vi "Set_Get_FVG.vi"(8 "error out":errorcluster, 9 "Tab Control":enum32{" START ", " HOME ", " TEST "}(ring), 10 "Message":T1=enum."Update Display", 11 "Enum":T2) -> (0 "error out 2":errorcluster, 2 "Tab Control 2":enum32{" START ", " HOME ", " TEST "}(ring), 3 "Message 2":T1)   [LabVIEW 2021]
uses:
  Control/Set_Get.ctl
  controls/test_sequence .ctl
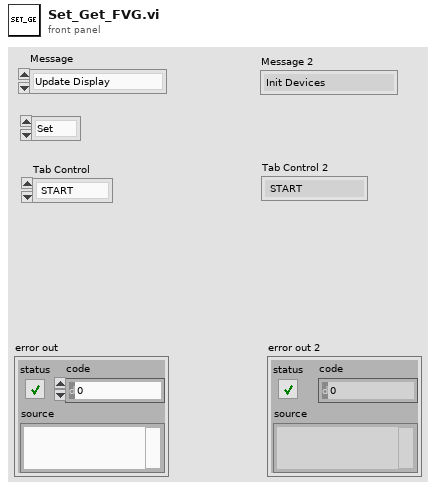
[diagram p1: front panel]
types:
  T1 = typedef "test_sequence .ctl" = enum16{"Init Devices", "Login", "Option Window", "Idle state", "Check", "Uncheck", "Scan Barcode", "Clear the test Containers", "Init-Pre Test", "Test ", "Result", "Report", "Database", "Update Display", "Confirm Quit", "Error", "Exit"}
  T2 = typedef "Set_Get.ctl" = enum16{"Set", "Get"}
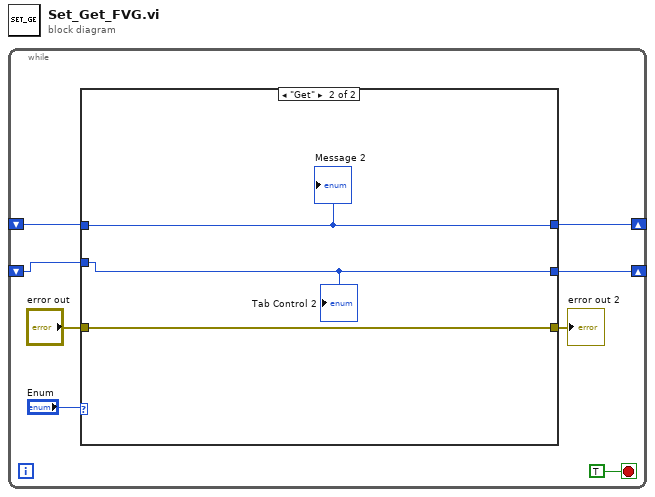
[diagram p0: block diagram]
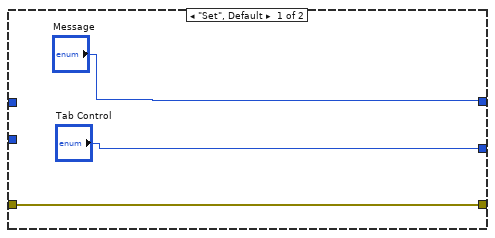
[diagram p2: hidden frame]
diagram:
  n1 = while {
    shift-right: [w7] -> _
    shift-left: _ -> [w6]
    shift-right: [w2] -> _
    shift-left: _ -> [w1]
    stop <- TRUE stop-if-true
    n2 = case shown="\"Get\"" "Enum" {
      tunnel: ["Message" w14] -> w7
      tunnel: w6 -> [_ w14]
      tunnel: [w10 w13] -> w3
      tunnel: "error out" -> [w10 w13]
      tunnel: ["Tab Control" w12] -> w2
      tunnel: w1 -> [_ w12]
      frame "Set", Default {
      }
      frame "Get" {
        "Message 2" <- w14
        "Tab Control 2" <- w12
      }
    }
    "error out 2" <- w3
  }
